vi "Check Packet Length.vi"(8 "error in (no error)":errorcluster, 10 "Mode":T1, 11 "payload in":u8[](array[numeric]) format="%.0x") -> (0 "error out":errorcluster, 3 "payload out":u8[](array[numeric]) format="%.0x")   [LabVIEW 2021, in "XNET CAN RW.lvclass"]
uses:
  XNET CAN RW.lvclass
  <vilib>/CIF Foundation/CIF CAN RW Core/typedef/CAN Mode.ctl
  typedef/Errors.ctl
  Add Error Core.vi
  <vilib>/CIF Foundation/CIF CAN RW Core/CAN_RW_CORE.lvclass
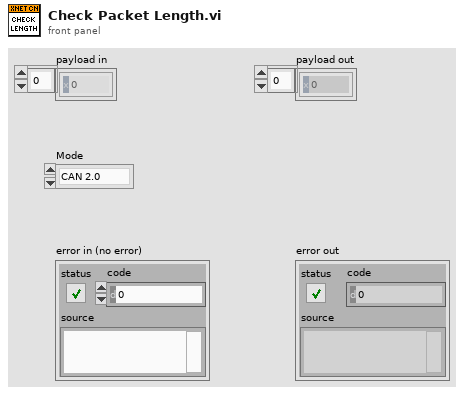
[diagram p1: front panel]
types:
  T1 = typedef "CAN_RW_CORE.lvclass/CAN Mode.ctl" = enum16{"CAN 2.0", "CAN FD"}
  T2 = typedef "XNET CAN RW.lvclass/Errors.ctl" = enum16{"TX Timeout", "Packet Length", "Invalid Start Time"}
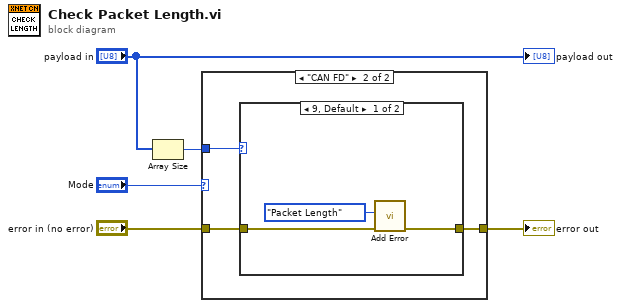
[diagram p0: block diagram]
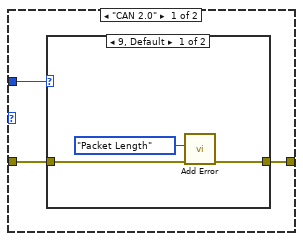
[diagram p2: hidden frame]
diagram:
  n1 = Array Size(array="payload in") -> (size(s)=w3:i32)
  n2 = case shown="\"CAN FD\"" "Mode" {
    tunnel: w3 -> [w8 w15]
    tunnel: "error in (no error)" -> [w7 w14]
    tunnel: [w6 w13] -> w1
    frame "CAN 2.0" {
      n3 = case shown="9, Default" w8 {
        tunnel: w7 -> [w10 w12]
        tunnel: [w9 w12] -> w6
        frame 9, Default {
          n4 = call "Add Error.vi"("error in (no error)"=w10, "Error"=Errors."Packet Length") -> ("error out"=w9:errorcluster)  [unwired: 9 in]
        }
        frame 0..8 {
        }
      }
    }
    frame "CAN FD" {
      n5 = case shown="9, Default" w15 {
        tunnel: w14 -> [w18 w19]
        tunnel: [w17 w19] -> w13
        frame 9, Default {
          n6 = call "Add Error.vi"("error in (no error)"=w18, "Error"=Errors."Packet Length") -> ("error out"=w17:errorcluster)  [unwired: 9 in]
        }
        frame 0..8, 12, 16, 20, 24, 32, 48, 64 {
        }
      }
    }
  }
  "error out" <- w1
  "payload out" <- "payload in"
